vi "INI-FGV.vi"(4 "Raw String? (F)":bool, 5 "Write If not found?":bool, 6 "Enum":T3, 7 "Prefered Section":string, 8 "error IN":errorcluster, 9 "Path":path, 10 ">> Default Value >>":string, 11 ">> Variable Name >>":string) -> (0 "error out":errorcluster, 1 "INIConfig":T1, 2 "Key?":bool, 3 "Array":string[](array[string]))   [LabVIEW 2017, in "INI-Static-Variable-Support.lvlib"]
uses:
  INI-Static-Variable-Support.lvlib
  _fgv-oper.ctl
  LabVIEW-Config/Config.ctl
  LabVIEW-Config/LineToken.ctl
  <userlib>/_NEVSTOP/Communicable State Machine(CSM)/_Support/ChangeFlag/ChangeFlag-Write.vi
  <userlib>/_NEVSTOP/Communicable State Machine(CSM)/Utility/Random Change Flag.vi
  <userlib>/_NEVSTOP/Communicable State Machine(CSM)/_Support/ChangeFlag/ChangeFlagDB.vi
  _Def-Ini-Variable.ctl
  CSMSVMgr/CSM-Static-Variable-Manager.lvclass
  LabVIEW-Config/LabVIEW-Config.lvlib
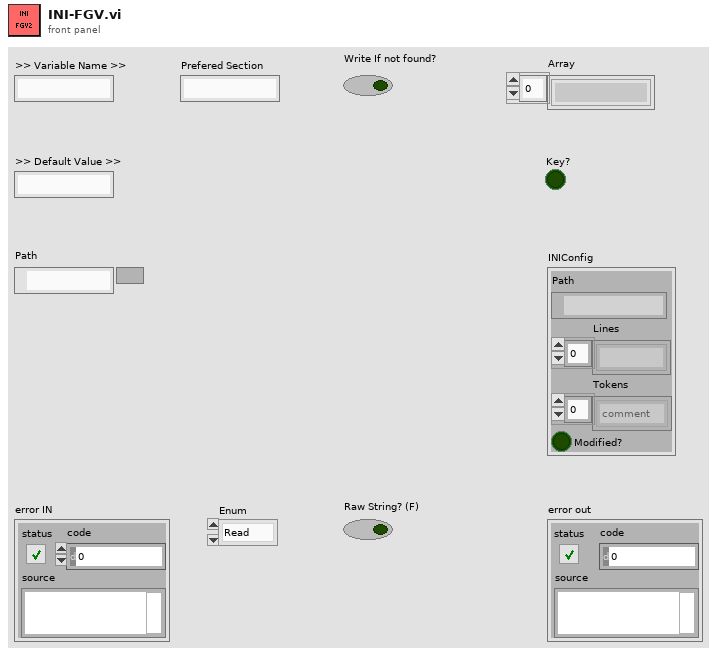
[diagram p1: front panel]
types:
  T1 = typedef "LabVIEW-Config.lvlib/Config.ctl" = cluster{"Path":path, "Lines":string[], "Tokens":T2[], "Modified?":bool}
  T2 = typedef "LabVIEW-Config.lvlib/LineToken.ctl" = enum8{"comment", "section", "key", "more"}
  T3 = typedef "INI-Static-Variable-Support.lvlib/_fgv-oper.ctl" = enum16{"Read", "Write", "Sync", "Sessions", "List Keys", "Load", "List Files", "List Variables", "List Permanent Variables", "Mark Temp Variable as Permenent", "unload", "INIConfig(Memory)", "Reset", "Restore Variable Value", "Load From String"}
  T4 = typedef "INI-Static-Variable-Support.lvlib/_Def-Ini-Variable.ctl" = cluster{"Variable Name":string, "Preferred Section":string}
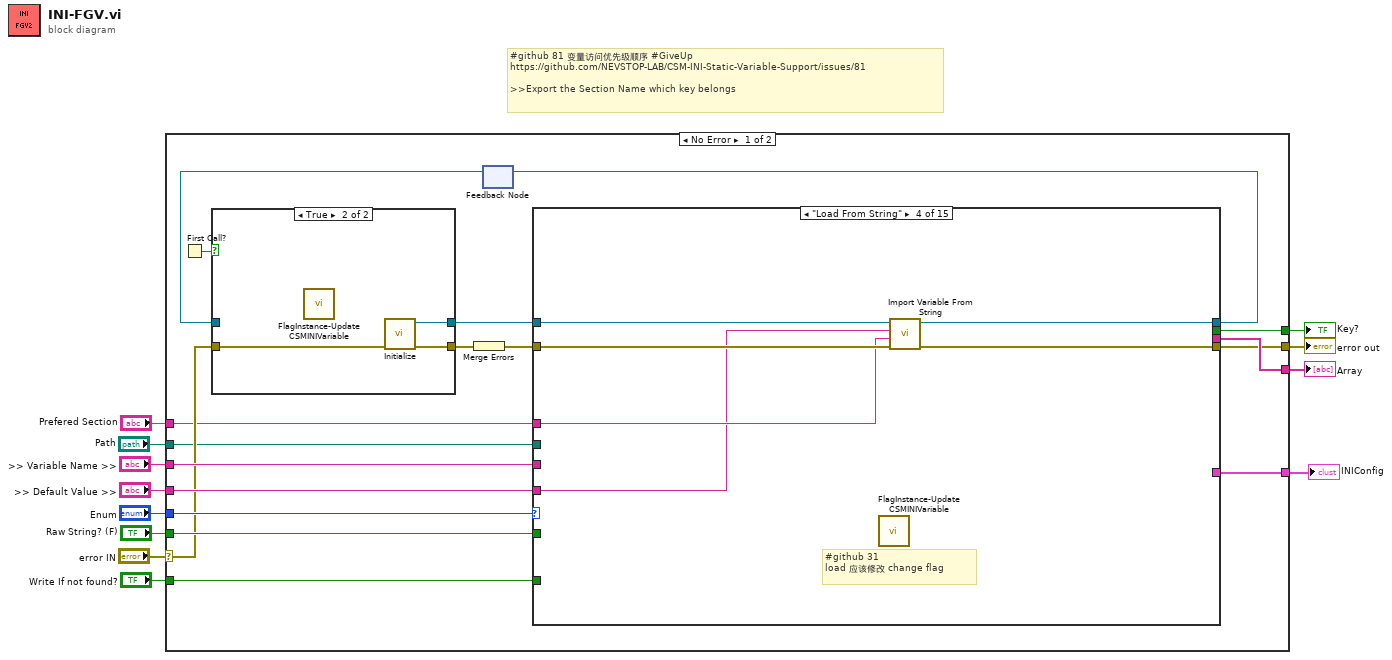
[diagram p0: block diagram]
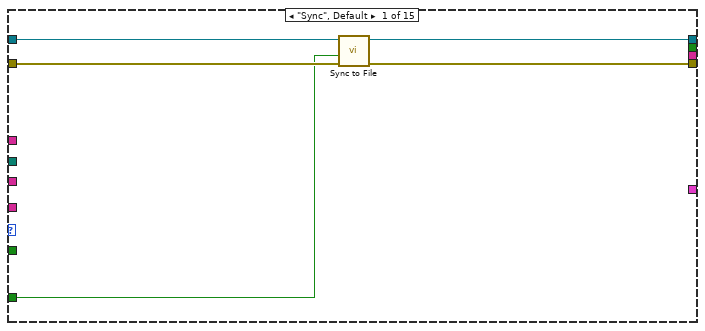
[diagram p2: hidden frame]
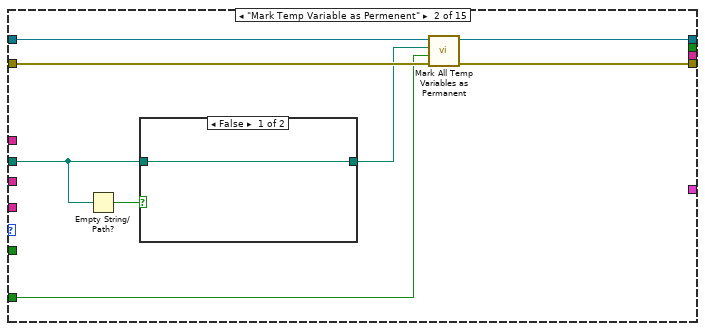
[diagram p3: hidden frame]
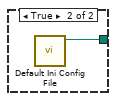
[diagram p4: hidden frame]
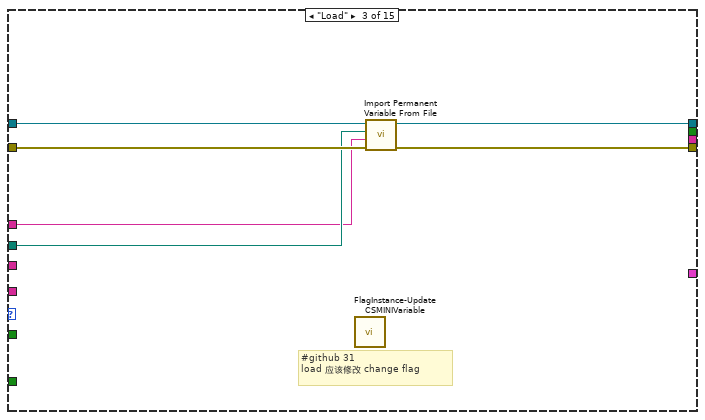
[diagram p5: hidden frame]
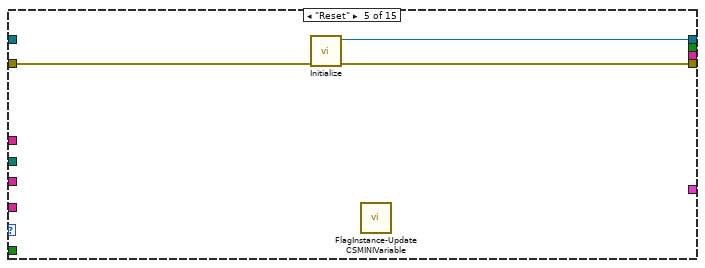
[diagram p6: hidden frame]
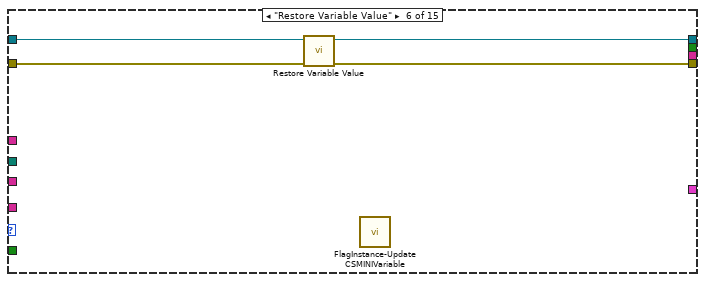
[diagram p7: hidden frame]
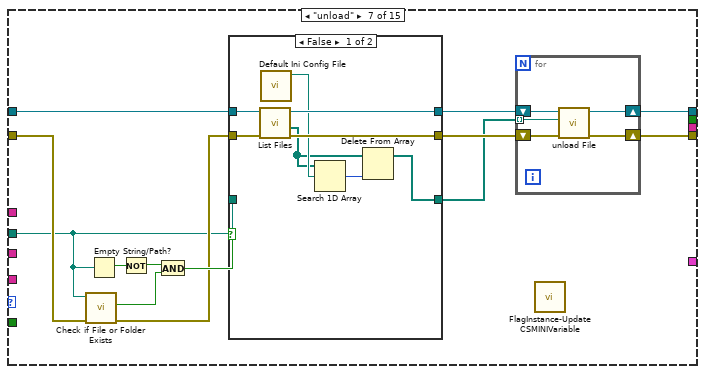
[diagram p8: hidden frame]
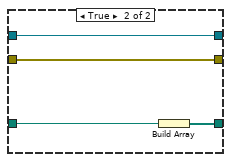
[diagram p9: hidden frame]
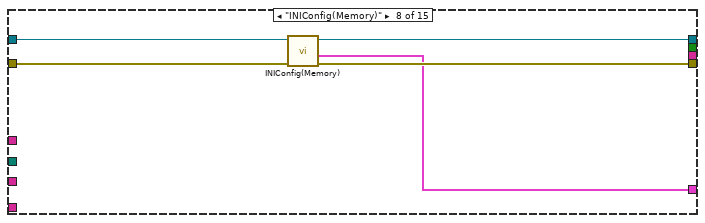
[diagram p10: hidden frame]
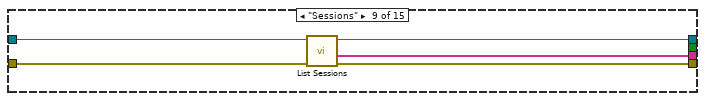
[diagram p11: hidden frame]
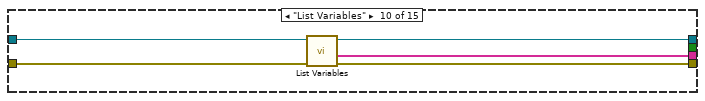
[diagram p12: hidden frame]
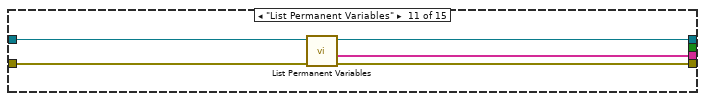
[diagram p13: hidden frame]
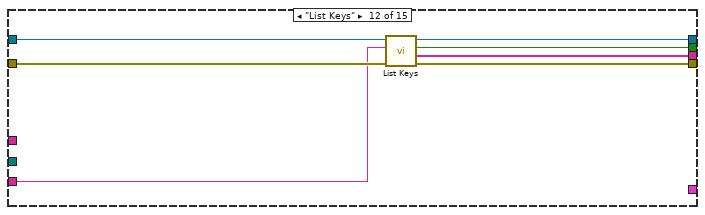
[diagram p14: hidden frame]
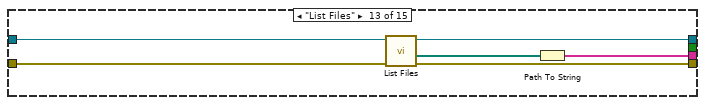
[diagram p15: hidden frame]
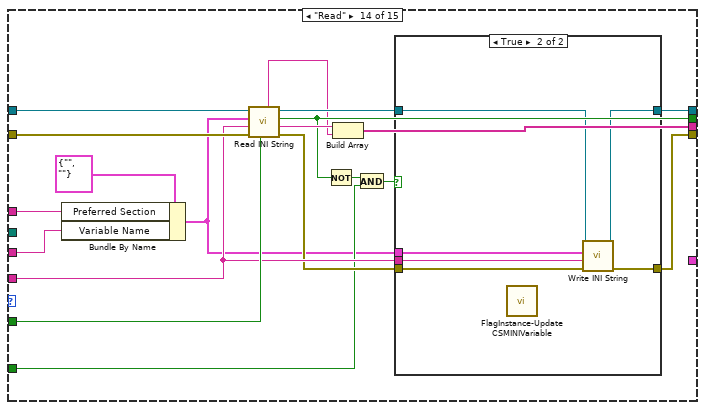
[diagram p16: hidden frame]
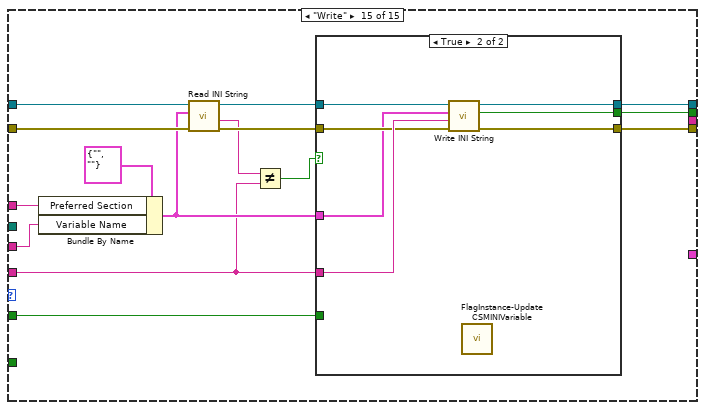
[diagram p18: hidden frame]
diagram:
  # "#github 81 变量访问优先级顺序 #GiveUp\nhttps://github.com/NEVSTOP-LAB/CSM-INI-Static-Variable-Support/issues/81\n\n>>Export the Section Name which key belongs"
  n1 = case shown="No Error" "error IN" {
    selector: "error IN" -> [w17 w184]
    tunnel: [w28 _] -> w12
    tunnel: ">> Default Value >>" -> [w27 _]
    tunnel: ">> Variable Name >>" -> [w26 _]
    tunnel: [w25 w184] -> w9
    tunnel: "Enum" -> [w20 _]
    tunnel: [w19 _] -> w7
    tunnel: "Raw String? (F)" -> [w18 _]
    tunnel: "Write If not found?" -> [w16 _]
    tunnel: "Path" -> [w15 _]
    tunnel: [w14 _] -> w2
    tunnel: "Prefered Section" -> [w13 _]
    frame No Error {
      n2 = First Call?() -> (First Call?: T/F=w24:bool)
      n3 = feedback #1() -> (w21:refnum<class "CSM-Static-Variable-Manager.lvclass">)  [unwired: 1 in]
      n4 = case shown="True" w24 {
        tunnel: [w180 w183] -> w29
        tunnel: [w179 w181] -> w23
        tunnel: w21 -> [w180 _]
        tunnel: w17 -> [w179 w182]
        frame False {
        }
        frame True {
          n5 = call "FlagInstance-Update CSMINIVariable.vi"() -> ()  [unwired: 10 in, 2 out]
          n6 = call "Initialize.vi"("Error in"=w182) -> ("Error out"=w181:errorcluster, "INI-Static-Variable-Support.lvlib:CSM-Static-Variable-Manager.lvclass"=w183:refnum<class "CSM-Static-Variable-Manager.lvclass">)  [unwired: 9 in]
        }
      }
      n7 = Merge Errors(w23) -> (w30:errorcluster)
      n8 = case shown="\"Load From String\"" w20 {
        tunnel: w30 -> [w32 w40 w48 w54 w60 w63 w68 w99 w100 w105 w110 w119 w125 w146 w166]
        tunnel: w29 -> [w35 w43 w51 w57 _ w64 w75 w97 w101 w106 w111 w117 w124 w134 w161]
        tunnel: [_ _ _ _ _ _ _ _ w102 w107 w112 w120 w122 w135 _] -> w28
        tunnel: w27 -> [_ _ _ w52 _ _ _ _ _ _ _ _ _ w142 w155]
        tunnel: w26 -> [_ _ _ _ _ _ _ _ _ _ _ w115 _ w131 w157]
        tunnel: [w33 w41 w49 w55 w59 w61 w76 w98 w103 w108 w113 w121 w127 w140 w169] -> w25
        tunnel: [w34 w42 w50 w56 w58 w62 w77 w96 w104 w109 w114 w116 w123 w133 w160] -> w22
        tunnel: [_ _ _ _ _ _ _ _ _ _ _ w118 _ w138 w168] -> w19
        tunnel: w18 -> [_ _ _ _ _ _ _ _ _ _ _ _ _ w144 w167]
        tunnel: w16 -> [w31 w36 _ _ _ _ _ _ _ _ _ _ _ w136 _]
        tunnel: w15 -> [_ w38 w47 _ _ _ w65 _ _ _ _ _ _ _ _]
        tunnel: [_ _ _ _ _ _ _ w95 _ _ _ _ _ _ _] -> w14
        tunnel: w13 -> [_ _ w46 w53 _ _ _ _ _ _ _ _ _ w130 w158]
        frame "Sync", Default {
          n9 = call "Sync to File.vi"("error in (no error)"=w32, "Write Reference?(F)"=w31, "CSM-Static-Variable-Manager in"=w35) -> ("error out"=w33:errorcluster, "CSM-Static-Variable-Manager out"=w34:refnum<class "CSM-Static-Variable-Manager.lvclass">)  [unwired: 7 in]
        }
        frame "Mark Temp Variable as Permenent" {
          n10 = Empty String/Path?(string/path=w38) -> (empty?=w39:bool)
          n11 = case shown="False" w39 {
            tunnel: w38 -> [w44 _]
            tunnel: [w44 w45] -> w37
            frame False {
            }
            frame True {
              n12 = call "Default Ini Config File.vi"() -> ("appended path"=w45:path)  [unwired: 11 in]
            }
          }
          n13 = call "Mark All Temp Variables as Permanent.vi"("error in (no error)"=w40, "SyncRef?(F)"=w36, "Path"=w37, "CSM-Static-Variable-Manager in"=w43) -> ("error out"=w41:errorcluster, "CSM-Static-Variable-Manager out"=w42:refnum<class "CSM-Static-Variable-Manager.lvclass">)  [unwired: 6 in]
        }
        frame "Load" {
          # "#github 31\nload 应该修改 change flag"
          n14 = call "FlagInstance-Update CSMINIVariable.vi"() -> ()  [unwired: 10 in, 2 out]
          n15 = call "Import Permanent Variable From File.vi"("error in (no error)"=w48, "section postfix"=w46, "Path"=w47, "CSM-Static-Variable-Manager in"=w51) -> ("error out"=w49:errorcluster, "CSM-Static-Variable-Manager out"=w50:refnum<class "CSM-Static-Variable-Manager.lvclass">)  [unwired: 6 in]
        }
        frame "Load From String" {
          # "#github 31\nload 应该修改 change flag"
          n16 = call "FlagInstance-Update CSMINIVariable.vi"() -> ()  [unwired: 10 in, 2 out]
          n17 = call "Import Variable From String.vi"("error in (no error)"=w54, "section postfix"=w53, "Configuration"=w52, "CSM-Static-Variable-Manager in"=w57) -> ("error out"=w55:errorcluster, "CSM-Static-Variable-Manager out"=w56:refnum<class "CSM-Static-Variable-Manager.lvclass">)  [unwired: 6 in]
        }
        frame "Reset" {
          n18 = call "Initialize.vi"("Error in"=w60) -> ("Error out"=w59:errorcluster, "INI-Static-Variable-Support.lvlib:CSM-Static-Variable-Manager.lvclass"=w58:refnum<class "CSM-Static-Variable-Manager.lvclass">)  [unwired: 9 in]
          n19 = call "FlagInstance-Update CSMINIVariable.vi"() -> ()  [unwired: 10 in, 2 out]
        }
        frame "Restore Variable Value" {
          n20 = call "Restore Variable Value.vi"("error in (no error)"=w63, "CSM-Static-Variable-Manager in"=w64) -> ("error out"=w61:errorcluster, "CSM-Static-Variable-Manager out"=w62:refnum<class "CSM-Static-Variable-Manager.lvclass">)  [unwired: 8 in]
          n21 = call "FlagInstance-Update CSMINIVariable.vi"() -> ()  [unwired: 10 in, 2 out]
        }
        frame "unload" {
          n22 = call <vilib>:"Check if File or Folder Exists.vi"("error in (no error)"=w68, "path"=w65) -> ("error out"=w67:errorcluster, "file or folder exists?"=w70:bool)  [unwired: 7 in, 1 out]
          n23 = Empty String/Path?(string/path=w65) -> (empty?=w72:bool)
          n24 = Not(x=w72) -> (.not. x?=w71:bool)
          n25 = And(x=w71, y=w70) -> (x .and. y?=w69:bool)
          n26 = case shown="False" w69 {
            tunnel: w75 -> [w85 w88]
            tunnel: [w84 w88] -> w74
            tunnel: [w83 w87] -> w73
            tunnel: w67 -> [w82 w87]
            tunnel: [w78 w86] -> w66
            tunnel: w65 -> [_ w89]
            frame False {
              n27 = call "List Files.vi"("error in (no error)"=w82, "CSM-Static-Variable-Manager in"=w85) -> ("error out"=w83:errorcluster, "File List"=w79:path[], "CSM-Static-Variable-Manager out"=w84:refnum<class "CSM-Static-Variable-Manager.lvclass">)  [unwired: 7 in]
              n28 = call "Default Ini Config File.vi"() -> ("appended path"=w81:path)  [unwired: 11 in]
              n29 = Search 1D Array(1D array=w79, element=w81) -> (index of element=w80:i32)  [unwired: 1 in]
              n30 = Delete From Array(array=w79, index=w80) -> (array with subset deleted=w78:path[])  [unwired: 1 in, 1 out]
            }
            frame True {
              n31 = Build Array(w89) -> (w86:path[])
            }
          }
          n32 = for {
            tunnel: w66 -> [w90] mode=indexing
            shift-right: [w94] -> w77
            shift-left: w74 -> [w92]
            shift-right: [w93] -> w76
            shift-left: w73 -> [w91]
            n33 = call "unload File.vi"("error in (no error)"=w91, "Path"=w90, "CSM-Static-Variable-Manager in"=w92) -> ("error out"=w93:errorcluster, "CSM-Static-Variable-Manager out"=w94:refnum<class "CSM-Static-Variable-Manager.lvclass">)  [unwired: 7 in]
          }
          n34 = call "FlagInstance-Update CSMINIVariable.vi"() -> ()  [unwired: 10 in, 2 out]
        }
        frame "INIConfig(Memory)" {
          n35 = call "INIConfig(Memory).vi"("error in (no error)"=w99, "CSM-Static-Variable-Manager in"=w97) -> ("error out"=w98:errorcluster, "Memory"=w95:T1, "CSM-Static-Variable-Manager out"=w96:refnum<class "CSM-Static-Variable-Manager.lvclass">)  [unwired: 7 in]
        }
        frame "Sessions" {
          n36 = call "List Sessions.vi"("error in (no error)"=w100, "CSM-Static-Variable-Manager in"=w101) -> ("error out"=w103:errorcluster, "Array"=w102:string[], "CSM-Static-Variable-Manager out"=w104:refnum<class "CSM-Static-Variable-Manager.lvclass">)  [unwired: 7 in]
        }
        frame "List Variables" {
          n37 = call "List Variables.vi"("error in (no error)"=w105, "CSM-Static-Variable-Manager in"=w106) -> ("error out"=w108:errorcluster, "Variables"=w107:string[], "CSM-Static-Variable-Manager out"=w109:refnum<class "CSM-Static-Variable-Manager.lvclass">)  [unwired: 7 in]
        }
        frame "List Permanent Variables" {
          n38 = call "List Permanent Variables.vi"("error in (no error)"=w110, "CSM-Static-Variable-Manager in"=w111) -> ("error out"=w113:errorcluster, "Permanent Variables"=w112:string[], "CSM-Static-Variable-Manager out"=w114:refnum<class "CSM-Static-Variable-Manager.lvclass">)  [unwired: 7 in]
        }
        frame "List Keys" {
          n39 = call "List Keys.vi"("error in (no error)"=w119, "Section Name"=w115, "CSM-Static-Variable-Manager in"=w117) -> ("error out"=w121:errorcluster, "Array"=w120:string[], "Key?"=w118:bool, "CSM-Static-Variable-Manager out"=w116:refnum<class "CSM-Static-Variable-Manager.lvclass">)  [unwired: 5 in]
        }
        frame "List Files" {
          n40 = call "List Files.vi"("error in (no error)"=w125, "CSM-Static-Variable-Manager in"=w124) -> ("error out"=w127:errorcluster, "File List"=w126:path[], "CSM-Static-Variable-Manager out"=w123:refnum<class "CSM-Static-Variable-Manager.lvclass">)  [unwired: 7 in]
          n41 = Path To String(path=w126) -> (string=w122:string[])
        }
        frame "Read" {
          n42 = Bundle By Name(cluster=T4 {"Variable Name"="", "Preferred Section"=""} ("Variable"), "Preferred Section"=w130, "Variable Name"=w131) -> (w129:T4)
          n43 = call "Read INI String.vi"("Force Default Session?(F)"=w144, "error in (no error)"=w146, "Default"=w142, "Variable"=w129, "CSM-Static-Variable-Manager in"=w134) -> ("error out"=w141:errorcluster, "Content"=w145:string, "Key Found?"=w138:bool, "CSM-Static-Variable-Manager out"=w143:refnum<class "CSM-Static-Variable-Manager.lvclass">, "Section Name"=w128:string)  [unwired: 2 in]
          n44 = Not(x=w138) -> (.not. x?=w137:bool)
          n45 = Build Array(w145, w128) -> (w135:string[])
          n46 = And(x=w137, y=w136) -> (x .and. y?=w139:bool)
          n47 = case shown="True" w139 {
            tunnel: w143 -> [w148 w149]
            tunnel: [w148 w154] -> w133
            tunnel: w129 -> [_ w153]
            tunnel: w142 -> [_ w152]
            tunnel: w141 -> [w147 w151]
            tunnel: [w147 w150] -> w140
            frame False {
            }
            frame True {
              n48 = call "FlagInstance-Update CSMINIVariable.vi"() -> ()  [unwired: 10 in, 2 out]
              n49 = call "Write INI String.vi"("error in (no error)"=w151, "Content"=w152, "Variable"=w153, "CSM-Static-Variable-Manager in"=w149) -> ("error out"=w150:errorcluster, "CSM-Static-Variable-Manager out"=w154:refnum<class "CSM-Static-Variable-Manager.lvclass">)  [unwired: 5 in, 1 out]
            }
          }
        }
        frame "Write" {
          n50 = Bundle By Name(cluster=T4 {"Variable Name"="", "Preferred Section"=""} ("Variable"), "Preferred Section"=w158, "Variable Name"=w157) -> (w156:T4)
          n51 = call "Read INI String.vi"("error in (no error)"=w166, "Variable"=w156, "CSM-Static-Variable-Manager in"=w161) -> ("error out"=w164:errorcluster, "Content"=w163:string, "CSM-Static-Variable-Manager out"=w165:refnum<class "CSM-Static-Variable-Manager.lvclass">)  [unwired: 4 in, 2 out]
          n52 = Not Equal?(x=w163, y=w155) -> (x != y?=w162:bool)
          n53 = case shown="True" w162 {
            tunnel: [w171 w178] -> w169
            tunnel: [w170 w177] -> w160
            tunnel: w155 -> [_ w176]
            tunnel: [_ w175] -> w168
            tunnel: w167 -> [_ _]
            tunnel: w165 -> [w170 w172]
            tunnel: w164 -> [w171 w174]
            tunnel: w156 -> [_ w173]
            frame False {
            }
            frame True {
              n54 = call "Write INI String.vi"("error in (no error)"=w174, "Content"=w176, "Variable"=w173, "CSM-Static-Variable-Manager in"=w172) -> ("error out"=w178:errorcluster, "Key Replaced?"=w175:bool, "CSM-Static-Variable-Manager out"=w177:refnum<class "CSM-Static-Variable-Manager.lvclass">)  [unwired: 5 in]
              n55 = call "FlagInstance-Update CSMINIVariable.vi"() -> ()  [unwired: 10 in, 2 out]
            }
          }
        }
      }
      n56 = feedback-in #1(w22) -> ()
    }
    frame Error {
    }
  }
  "Array" <- w12
  "error out" <- w9
  "Key?" <- w7
  "INIConfig" <- w2
